vi "SOS_Timer.vi"(0 "error in (no error)":errorcluster caption="错误输入（无错误）", 2 "Reset Timer":bool, 3 "Pressed":bool, 4 "Required Milliseconds":u32) -> (1 "error out":errorcluster caption="错误输出", 5 "Held Milliseconds":u32, 6 "SOS Requested":bool)   [LabVIEW 2020]
doc: "PLACEHOLDER: error interface only. Alarm simulation NOT implemented."
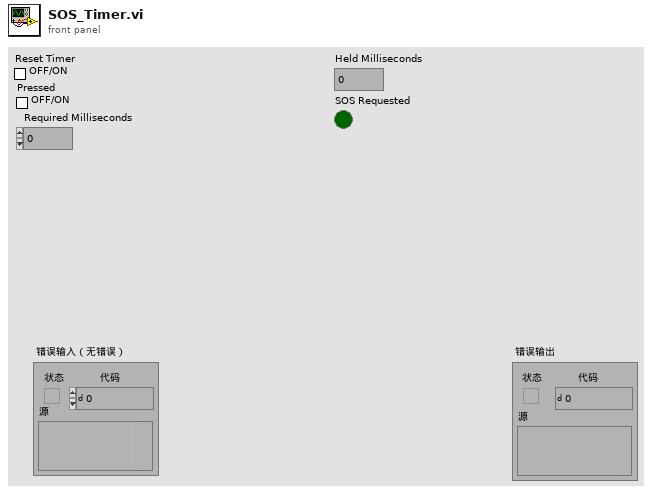
[diagram p1: front panel]
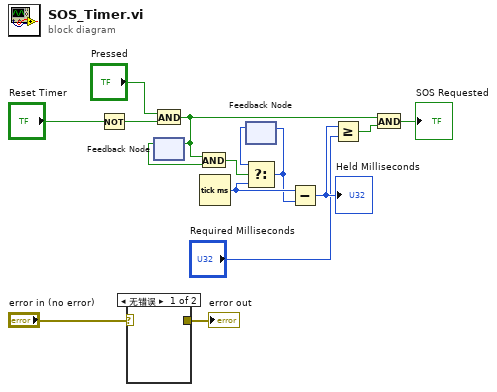
[diagram p0: block diagram]
diagram:
  n1 = Not(x="Reset Timer") -> (.not. x?=w12:bool)
  n2 = case shown="无错误" "error in (no error)" {
    selector: "error in (no error)" -> [_ w16]
    tunnel: [_ w16] -> w14
    frame No Error {
    }
    frame Error {
    }
  }
  "error out" <- w14
  n3 = And(x="Pressed", y=w12) -> (x .and. y?=w10:bool)
  n4 = feedback-in #1(w10) -> ()
  n5 = feedback #1() -> (w9:bool)  [unwired: 1 in]
  n6 = And(x=w10, y=w9) -> (x .and. y?=w8:bool)
  n7 = Tick Count (ms)() -> (millisecond timer value=w7:u32)
  n8 = feedback #2() -> (w6:u32)  [unwired: 1 in]
  n9 = Select(t=w6, s=w8, f=w7) -> (s? t:f=w5:u32)
  n10 = feedback-in #2(w5) -> ()
  n11 = Subtract(x=w7, y=w5) -> (x-y=w4:u32)
  "Held Milliseconds" <- w4
  n12 = Greater Or Equal?(x=w4, y="Required Milliseconds") -> (x >= y?=w2:bool)
  n13 = And(x=w10, y=w2) -> (x .and. y?=→"SOS Requested":bool)
